vi "GUI_CH1_Comm_Stream.vi"() -> ()   [LabVIEW 2018]
uses:
  Stream/Stream.lvclass
  RxTx/RxTx.lvclass
  Stream/Stream.lvclass/Stream.ctl
panel:
  out "error out 2":errorcluster
  out "error out":errorcluster
  in  "RxTx.lvclass 2":refnum<class "RxTx.lvclass">
  in  "Stream.lvclass 2":refnum<class "Stream.lvclass">
  in  "RxTx.lvclass":refnum<class "RxTx.lvclass">
  in  "Stream.lvclass":refnum<class "Stream.lvclass">
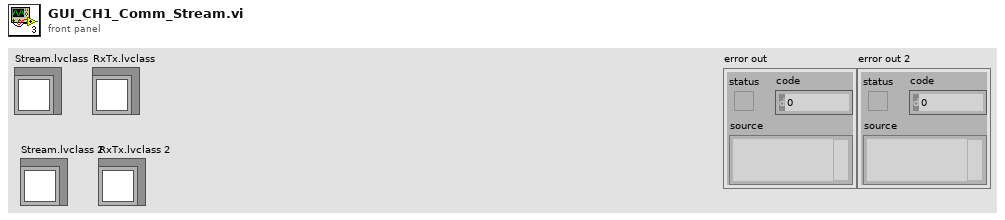
[diagram p1: front panel]
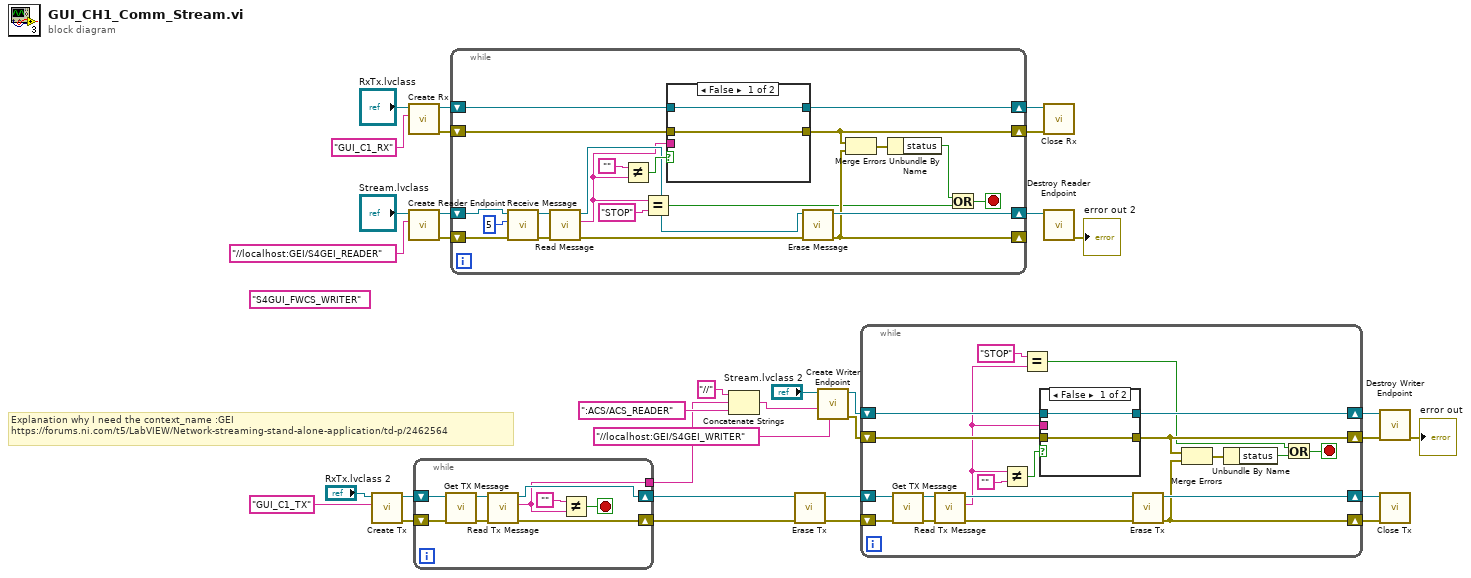
[diagram p0: block diagram]
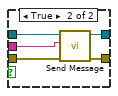
[diagram p2: hidden frame]
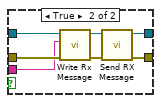
[diagram p3: hidden frame]
diagram:
  (unwired) "S4GUI_FWCS_WRITER" ("reader name")
  # "Explanation why I need the context_name :GEI\nhttps://forums.ni.com/t5/LabVIEW/Network-streaming-stand-alone-application/td-p/2462564"
  n1 = call "Create Tx.vi"("Writer Name"="GUI_C1_TX" ("Reader Name"), "RxTx in"="RxTx.lvclass 2") -> ("error out"=w8:errorcluster, "RxTx out"=w7:refnum<class "RxTx.lvclass">)  [unwired: 8 in]
  n2 = call "Create Rx.vi"("Reader Name"="GUI_C1_RX", "RxTx in"="RxTx.lvclass") -> ("error out"=w26:errorcluster, "RxTx out"=w27:refnum<class "RxTx.lvclass">)  [unwired: 8 in]
  n3 = call "Create Reader Endpoint.vi"("reader name"="//localhost:GEI/S4GEI_READER", "Stream in"="Stream.lvclass") -> ("error out"=w31:errorcluster, "Stream out"=w32:refnum<class "Stream.lvclass">)  [unwired: 8 in]
  n4 = while {
    shift-right: [w38] -> w11
    shift-left: w8 -> [w37]
    shift-right: [w36] -> w12
    shift-left: w7 -> [w35]
    tunnel: [w34] -> w5
    stop <- w39 stop-if-true
    n5 = call "Get TX Message.vi"("error in (no error)"=w37, "RxTx in"=w35) -> ("error out"=w41:errorcluster, "RxTx out"=w42:refnum<class "RxTx.lvclass">)  [unwired: 8 in]
    n6 = call "Read Tx Message.vi"("error in (no error)"=w41, "RxTx in"=w42) -> ("error out"=w38:errorcluster, "Tx Message"=w34:string, "RxTx out"=w36:refnum<class "RxTx.lvclass">)  [unwired: 7 in]
    n7 = Not Equal?(x="", y=w34) -> (x != y?=w39:bool)
  }
  n8 = while {
    shift-right: [w48] -> _
    shift-left: w31 -> [w62]
    shift-right: [w51] -> w30
    shift-left: w32 -> [w63]
    shift-right: [w55] -> w24
    shift-left: w26 -> [w59]
    shift-right: [w57] -> w25
    shift-left: w27 -> [w58]
    stop <- w45 stop-if-true
    n9 = call "Receive Message.vi"("error in (no error)"=w62, "timeout ms"=5, "Stream in"=w63) -> ("error out"=w60:errorcluster, "Stream out"=w61:refnum<class "Stream.lvclass">)  [unwired: 7 in]
    n10 = call "Read Message.vi"("error in (no error)"=w60, "Stream in"=w61) -> ("error out"=w50:errorcluster, "Message"=w47:string, "Stream out"=w49:refnum<class "Stream.lvclass">)  [unwired: 7 in]
    n11 = Not Equal?(x="", y=w47) -> (x != y?=w52:bool)
    n12 = Equal?(x=w47, y="STOP" ("reader name")) -> (x = y?=w43:bool)
    n13 = case shown="False" w52 {
      tunnel: w59 -> [w64 w70]
      tunnel: w58 -> [w65 w69]
      tunnel: w47 -> [_ w68]
      tunnel: [w65 w67] -> w57
      tunnel: [w64 w66] -> w55
      frame False {
      }
      frame True {
        n14 = call "Write Rx Message.vi"("error in (no error)"=w70, "Rx Message"=w68, "RxTx in"=w69) -> ("error out"=w71:errorcluster, "RxTx out"=w72:refnum<class "RxTx.lvclass">)  [unwired: 7 in]
        n15 = call "Send RX Message.vi"("error in (no error)"=w71, "RxTx in"=w72) -> ("error out"=w66:errorcluster, "RxTx out"=w67:refnum<class "RxTx.lvclass">)  [unwired: 8 in]
      }
    }
    n16 = call "Erase Message.vi"("error in (no error)"=w50, "Stream in"=w49) -> ("error out"=w48:errorcluster, "Stream out"=w51:refnum<class "Stream.lvclass">)  [unwired: 8 in]
    n17 = Merge Errors(w55, w48) -> (w56:errorcluster)
    n18 = Unbundle By Name(w56) -> ("status"=w44:bool)
    n19 = Or(x=w44, y=w43) -> (x .or. y?=w45:bool)
  }
  n20 = Concatenate Strings("//" ("reader name"), w5, ":ACS/ACS_READER" ("reader name")) -> (w3:string)
  n21 = call "Erase Tx.vi"("error in (no error)"=w11, "RxTx in"=w12) -> ("error out"=w9:errorcluster, "RxTx out"=w10:refnum<class "RxTx.lvclass">)  [unwired: 8 in]
  n22 = call "Create Writer Endpoint.vi"("writer name"="//localhost:GEI/S4GEI_WRITER" ("reader name"), "reader name"=w3, "Stream in"="Stream.lvclass 2") -> ("error out"=w16:errorcluster, "Stream out"=w18:refnum<class "Stream.lvclass">)  [unwired: 7 in]
  n23 = while {
    shift-right: [w84] -> w15
    shift-left: w16 -> [w86]
    shift-right: [w85] -> w22
    shift-left: w18 -> [w87]
    shift-right: [w79] -> w19
    shift-left: w9 -> [w88]
    shift-right: [w81] -> w20
    shift-left: w10 -> [w89]
    stop <- w76 stop-if-true
    n24 = call "Get TX Message.vi"("error in (no error)"=w88, "RxTx in"=w89) -> ("error out"=w91:errorcluster, "RxTx out"=w90:refnum<class "RxTx.lvclass">)  [unwired: 8 in]
    n25 = call "Read Tx Message.vi"("error in (no error)"=w91, "RxTx in"=w90) -> ("error out"=w80:errorcluster, "Tx Message"=w74:string, "RxTx out"=w82:refnum<class "RxTx.lvclass">)  [unwired: 7 in]
    n26 = Not Equal?(x=w74, y="") -> (x != y?=w73:bool)
    n27 = Equal?(x="STOP", y=w74) -> (x = y?=w78:bool)
    n28 = case shown="False" w73 {
      tunnel: w87 -> [w94 w99]
      tunnel: w86 -> [w93 w98]
      tunnel: [w94 w97] -> w85
      tunnel: w74 -> [_ w96]
      tunnel: [w93 w95] -> w84
      frame False {
      }
      frame True {
        n29 = call "Send Message.vi"("error in (no error)"=w98, "Message"=w96, "Stream in"=w99) -> ("error out"=w95:errorcluster, "Stream out"=w97:refnum<class "Stream.lvclass">)  [unwired: 7 in]
      }
    }
    n30 = call "Erase Tx.vi"("error in (no error)"=w80, "RxTx in"=w82) -> ("error out"=w79:errorcluster, "RxTx out"=w81:refnum<class "RxTx.lvclass">)  [unwired: 8 in]
    n31 = Merge Errors(w84, w79) -> (w92:errorcluster)
    n32 = Unbundle By Name(w92) -> ("status"=w77:bool)
    n33 = Or(x=w78, y=w77) -> (x .or. y?=w76:bool)
  }
  n34 = call "Close Rx.vi"("error in (no error)"=w24, "RxTx in"=w25) -> ()  [unwired: 8 in, 2 out]
  n35 = call "Destroy Reader Endpoint.vi"("Stream in"=w30) -> ("error out"=→"error out 2":errorcluster)  [unwired: 9 in, 1 out]
  n36 = call "Destroy Writer Endpoint.vi"("error in (no error)"=w15, "Stream in"=w22) -> ("error out"=→"error out":errorcluster)  [unwired: 8 in, 1 out]
  n37 = call "Close Tx.vi"("error in (no error)"=w19, "RxTx in"=w20) -> ()  [unwired: 8 in, 2 out]
